vi "MQTT Reason DISCONNECT.vi"(10 "Disconnect Reason Code":T1 items=[" Close the connection normally. Do not send the Will Message."=0, " The Client wishes to disconnect but requires that the Server also publishes its Will Message."=4, " The Connection is closed but the sender either does not wish to reveal the reason, or none of the other Reason Codes apply."=128, " The received packet does not conform to this specification."=129, " An unexpected or out of order packet was received."=130, " The packet received is valid but cannot be processed by this implementation."=131, " The request is not authorized."=135, " The Server is busy and cannot continue processing requests from this Client."=137, " The Server is shutting down."=139, " The Connection is closed because no packet has been received for 1.5 times the Keepalive time."=141, " Another Connection using the same ClientID has connected causing this Connection to be closed."=142, " The Topic Filter is correctly formed, but is not accepted by this Server."=143, " The Topic Name is correctly formed, but is not accepted by this Client or Server."=144, " The Client or Server has received more than Receive Maximum publication for which it has not sent PUBACK or PUBCOMP."=147, " The Client or Server has received a PUBLISH packet containing a Topic Alias which is greater than the Maximum Topic Alias it sent in the CONNECT or CONNACK packet."=148, " The packet size is greater than Maximum Packet Size for this Client or Server."=149, " The received data rate is too high."=150, " An implementation or administrative imposed limit has been exceeded."=151, " The Connection is closed due to an administrative action."=152, " The payload format does not match the one specified by the Payload Format Indicator."=153, " The Server has does not support retained messages."=154, " The Client specified a QoS greater than the QoS specified in a Maximum QoS in the CONNACK."=155, " The Client should temporarily change its Server."=156, " The Server is moved and the Client should permanently change its server location."=157, " The Server does not support Shared Subscriptions."=158, " This connection is closed because the connection rate is too high."=159, " The maximum connection time authorized for this connection has been exceeded."=160, " The Server does not support Subscription Identifiers; the subscription is not accepted."=161, " The Server does not support Wildcard Subscriptions; the subscription is not accepted."=162]) -> (3 "String":string)   [LabVIEW 2019, in "KoRE-MQTT.lvlib"]
doc: "Copyright (c) 2025 KoRElibs.com\nSPDX-License-Identifier: EUPL-1.2\n\nThis VI is licensed under the European Union Public License (EUPL) Version 1.2. You may use this VI unmodified in proprietary works. If you distribute a modified version of this file, the modified file must be released under the EUPL-1.2. Full license: https://joinup.ec.europa.eu/asset/eupl/eupl/1.2/"
uses:
  KoRE-MQTT.lvlib
  TypeDefs/MQTT Reason - Disconnect Type.ctl
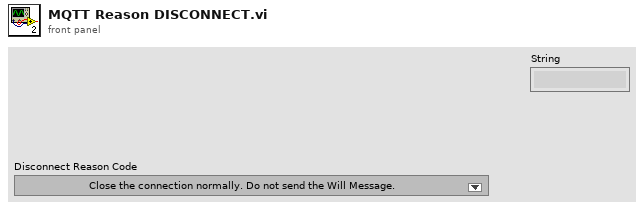
[diagram p1: front panel]
types:
  T1 = typedef "KoRE-MQTT.lvlib/MQTT Reason - Disconnect Type.ctl" = u16
  T2 = typedef "LVStringsAndValuesArrayTypeDef_U16.ctl" = cluster{"String":string, "Value":u16}[]
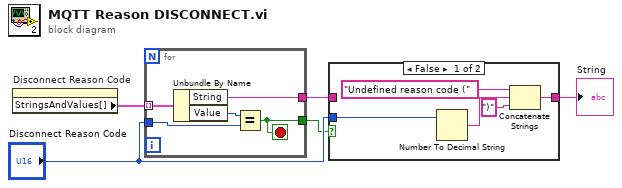
[diagram p0: block diagram]
diagram:
  n1 = property on="Disconnect Reason Code" class="Ring (strict)"() -> ("StringsAndValues[]"=w1:T2)  [unwired: 2 in, 2 out]
  n2 = for {
    tunnel: w1 -> [w10] mode=indexing
    tunnel: "Disconnect Reason Code" -> [w8]
    tunnel: [w7] -> w3
    tunnel: [w6] -> w2
    stop <- w6 stop-if-true
    n3 = Unbundle By Name(w10) -> ("String"=w7:string, "Value"=w9:u16)
    n4 = Equal?(x=w9, y=w8) -> (x = y?=w6:bool)
  }
  n5 = case shown="False" w2 {
    tunnel: [w14 w16] -> w4
    tunnel: w3 -> [_ w16]
    tunnel: "Disconnect Reason Code" -> [w15 _]
    frame False {
      n6 = Number To Decimal String(number=w15) -> (decimal integer string=w12:string)  [unwired: 1 in]
      n7 = Concatenate Strings("Undefined reason code (" ("string"), w12, ")" ("string")) -> (w14:string)
    }
    frame True {
    }
  }
  "String" <- w4
